vi "Filter PolyVI Instance VI Paths.vi"(11 "VI Paths":path[](array[path])) -> (3 "VI Paths out":path[](array[path]))   [LabVIEW 2014, in "VIHelpeksAPI.lvlib"]
doc: "::: VI Helpeks :::\nCopyright (c) 2000-2026 Konstantin Shifershteyn. All rights reserved."
uses:
  VIHelpeksAPI.lvlib
panel:
  # "VI Helpeks\nCopyright (c) 2012-2026 Konstantin Shifershteyn"
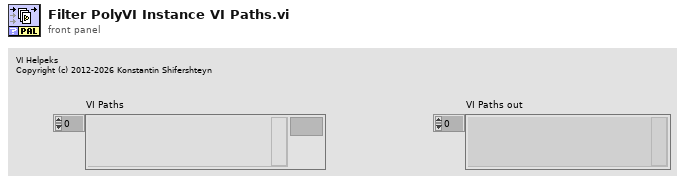
[diagram p1: front panel]
types:
  T1 = typedef "NI_FileType.lvlib/LVFileType.ctl" = enum32{"Invalid file", "Unknown type", "Instrument", "Control", "Polymorphic VI", "Project", "Library", "LVClass", "XControl", "XNode", "Shared library", ".NET assembly", "ActiveX interface", "CIN", "Run-time menu", "Palette menu", "Help file", "LLB", "XNode Edit Dependency", "Class Private Data Control", "Statechart", "MathScript .m file", "Ladder Diagram", "LVLibp", "XNode Build Dependency"}
  T2 = cluster{"path":path, "delimited name":string, "type":T1, "iState":u32, "iStyle":u16, "wStyle":u16, "buttons":u16, "viflags":u32, "viflags2":u32, "links":u32[]}[]
  T3 = cluster{"path":path, "delimited name":string, "type":T1, "iState":u32, "iStyle":u16, "wStyle":u16, "buttons":u16, "viflags":u32, "viflags2":u32, "links":u32[]}
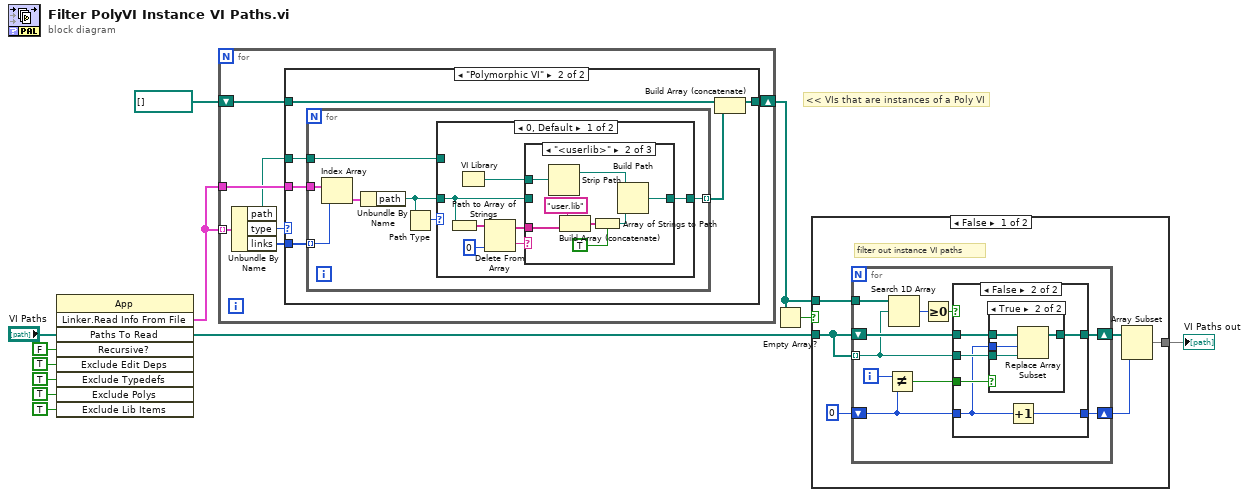
[diagram p0: block diagram]
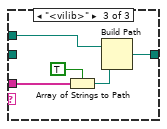
[diagram p7: hidden frame]
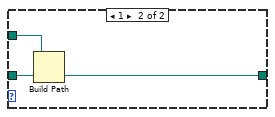
[diagram p8: hidden frame]
diagram:
  # "<< VIs that are instances of a Poly VI"
  n1 = invoke class="App" method="Linker.Read Info From File"("Paths To Read"="VI Paths", "Recursive?"=FALSE, "Exclude Edit Deps"=TRUE ("Exclude Edit Time Dependencies"), "Exclude Typedefs"=TRUE, "Exclude Polys"=TRUE ("Exclude Poly VIs"), "Exclude Lib Items"=TRUE ("Exclude Unused Library Items")) -> ("Linker.Read Info From File"=w6:T2)  [unwired: 3 in, 8 out]
  n2 = for {
    tunnel: w6 -> [w18] mode=indexing
    tunnel: w6 -> [w15]
    shift-right: [w13] -> w1
    shift-left: path[] [] -> [w14]
    n3 = Unbundle By Name(w18) -> ("path"=w12:path, "type"=w17:T1, "links"=w16:u32[])
    n4 = case shown="\"Polymorphic VI\"" w17 {
      tunnel: w16 -> [_ w25]
      tunnel: w15 -> [_ w24]
      tunnel: w14 -> [w19 w22]
      tunnel: [w19 w21] -> w13
      tunnel: w12 -> [_ w20]
      frame Default {
      }
      frame "Polymorphic VI" {
        n5 = for {
          tunnel: w25 -> [w31] mode=indexing
          tunnel: w24 -> [w32]
          tunnel: [w26] -> w23 mode=indexing
          tunnel: w20 -> [w27]
          n6 = Index Array(array=w32, index=w31) -> (element=w30:T3)
          n7 = Unbundle By Name(w30) -> ("path"=w28:path)
          n8 = Path Type(1:w28) -> (0:w29:i16)
          n9 = case shown="0, Default" w29 {
            tunnel: w28 -> [w36 w56]
            tunnel: w27 -> [_ w55]
            tunnel: [w35 w54] -> w26
            frame 0, Default {
              n10 = Path to Array of Strings(0:w36) -> (2:w39:string[])  [unwired: 1 out]
              n11 = VI Library() -> (path=w33:path)
              n12 = Delete From Array(array=w39, index=0) -> (deleted portion=w37:string, array with subset deleted=w34:string[])  [unwired: 1 in]
              n13 = case shown="\"<userlib>\"" w37 {
                tunnel: w36 -> [w40 _ _]
                tunnel: [w40 w48 w53] -> w35
                tunnel: w34 -> [_ w47 w50]
                tunnel: w33 -> [_ w42 w49]
                frame Default {
                }
                frame "<userlib>" {
                  n14 = Strip Path(path=w42) -> (stripped path=w41:path)  [unwired: 1 out]
                  n15 = Build Array (concatenate)("user.lib", w47) -> (w46:string[])
                  n16 = Array of Strings to Path(0:w46, 1:TRUE) -> (2:w45:path)
                  n17 = Build Path(base path=w41, name or relative path=w45) -> (appended path=w48:path)
                }
                frame "<vilib>" {
                  n18 = Array of Strings to Path(0:w50, 1:TRUE) -> (2:w52:path)
                  n19 = Build Path(base path=w49, name or relative path=w52) -> (appended path=w53:path)
                }
              }
            }
            frame 1 {
              n20 = Build Path(base path=w55, name or relative path=w56) -> (appended path=w54:path)
            }
          }
        }
        n21 = Build Array (concatenate)(w22, w23) -> (w21:path[])
      }
    }
  }
  n22 = Empty Array?(array=w1) -> (empty?=w2:bool)
  n23 = case shown="False" w2 {
    tunnel: "VI Paths" -> [w60 w86]
    tunnel: [w58 w86] -> w3
    tunnel: w1 -> [w57 _]
    frame False {
      # "filter out instance VI paths"
      n24 = for {
        tunnel: w57 -> [w72]
        shift-right: [w68] -> w61
        shift-left: w60 -> [w71]
        tunnel: w60 -> [w70] mode=indexing
        shift-right: [w69] -> w59
        shift-left: 0 -> [w65]
        i -> [w66]
        n25 = Not Equal?(x=w66, y=w65) -> (x != y?=w67:bool)
        n26 = Search 1D Array(1D array=w72, element=w70) -> (index of element=w64:i32)  [unwired: 1 out]
        n27 = Greater Or Equal To 0?(x=w64) -> (x >= 0?=w63:bool)
        n28 = case shown="False" w63 {
          tunnel: w71 -> [w74 w80]
          tunnel: w70 -> [_ w79]
          tunnel: w65 -> [w73 w76]
          tunnel: [w73 w75] -> w69
          tunnel: [w74 w78] -> w68
          tunnel: w67 -> [_ w77]
          frame True {
          }
          frame False {
            n29 = case shown="True" w77 {
              tunnel: w80 -> [w81 w85]
              tunnel: w79 -> [_ w84]
              tunnel: [w81 w83] -> w78
              tunnel: w76 -> [_ w82]
              frame False {
              }
              frame True {
                n30 = Replace Array Subset(array=w85, new element=w84, index=w82) -> (w83:path[])
              }
            }
            n31 = Increment(x=w76) -> (x+1=w75:i32)
          }
        }
      }
      n32 = Array Subset(array=w61, length=w59) -> (w58:path[])  [unwired: 1 in]
    }
    frame True {
    }
  }
  "VI Paths out" <- w3
